vi "P10 Timestamp Survival.vi"() -> ()   [LabVIEW 2026]
doc: "Round 11 probe. Three constants of three types wired straight to three indicators, so one convert+export answers two questions at once: (a) is a non-empty timestamp literal discarded, (b) does the same document keep its string and double literals. Every literal is unique so a stale file cannot fake a pass."
panel:
  out "Num Out":dbl
  out "Str Out":string
  out "Ts Out":timestamp
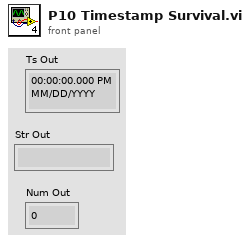
[diagram p1: front panel]
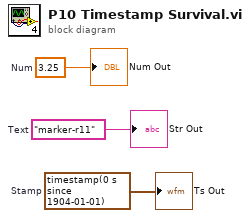
[diagram p0: block diagram]
diagram:
  w1 = 3.25  # Num
  w2 = "marker-r11"  # Text
  w3 = timestamp(0 s since 1904-01-01)  # Stamp
  "Ts Out" <- w3
  "Str Out" <- w2
  "Num Out" <- w1
